vi "PathPlanner_PathConstraints_GetAll.vi"(11 "PathPlannerConstraints":T1={"MaxVelocityMps;"=0.0, "MaxAccelerationMpsSq;"=0.0, "MaxAngularVelRadPsEc;"=0.0, "MaxAngularAccRadPSecSq"=0.0, "Exists"=FALSE, "Unlimited"=FALSE, "NominalVoltageVolts"=12.0}) -> (0 "MaxAngularAccRadPSecSq":dbl, 1 "MaxAngularVelRadPsEc;":dbl, 2 "MaxAccelerationMpsSq;":dbl, 3 "MaxVelocityMps;":dbl, 4 "Exists":bool)   [LabVIEW 2019, in "PathPlanner24.lvlib"]
doc: "Get all elements of Path Constraints cluster\n\nInputs:\n - PathConstraint - cluster - The path constraints to query\n\nOutputs:\n - maxVelocityMps - double - Max linear velocity (M/S)\n - maxAccelerationMpsSq - double - Max linear acceleration (M/S^2)\n - maxAngularVelocityRps - double - Max angular velocity (Rad/S)\n - maxAngularAccelerationRpsSq - double - Max angular acceleration (Rad/S^2)\n - exists - boolean - TRUE if this data cluster is not null."
uses:
  PathPlanner24.lvlib
  TypeDef/PathPlannerPathConstraints.ctl
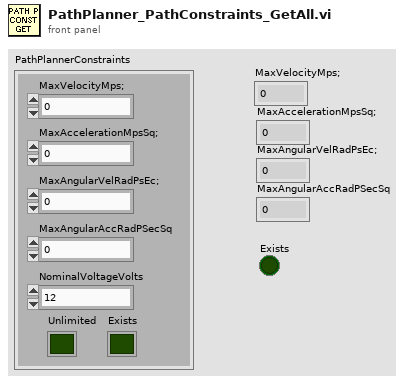
[diagram p1: front panel]
types:
  T1 = typedef "PathPlanner24.lvlib/PathPlannerPathConstraints.ctl" = cluster{"MaxVelocityMps;":dbl, "MaxAccelerationMpsSq;":dbl, "MaxAngularVelRadPsEc;":dbl, "MaxAngularAccRadPSecSq":dbl, "Exists":bool, "Unlimited":bool, "NominalVoltageVolts":dbl}
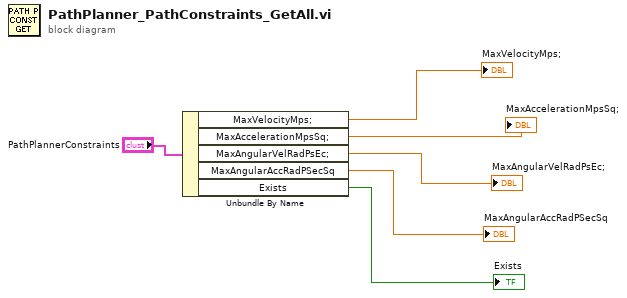
[diagram p0: block diagram]
diagram:
  n1 = Unbundle By Name("PathPlannerConstraints") -> ("MaxVelocityMps;"=→"MaxVelocityMps;":dbl, "MaxAccelerationMpsSq;"=→"MaxAccelerationMpsSq;":dbl, "MaxAngularVelRadPsEc;"=→"MaxAngularVelRadPsEc;":dbl, "MaxAngularAccRadPSecSq"=→"MaxAngularAccRadPSecSq":dbl, "Exists"=→"Exists":bool)
